vi "Convert Press. Regul. Sensor V to Bar.vi"(11 "V. Regulator Press. Sensor":dbl) -> (3 "Press. at Regulator (Bar)":dbl)   [LabVIEW 2024]
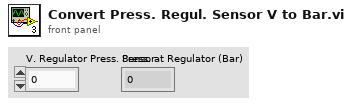
[diagram p1: front panel]
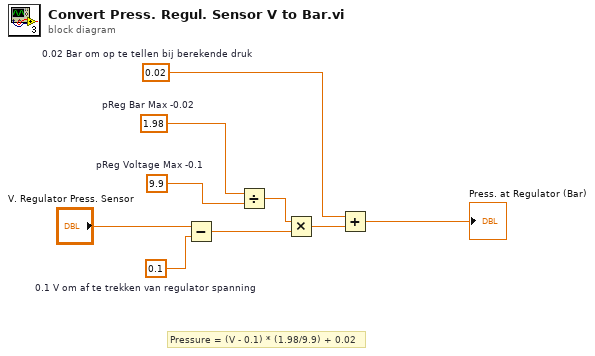
[diagram p0: block diagram]
diagram:
  w7 = 0.02  # 0.02 Bar om op te tellen bij berekende druk
  w4 = 9.9  # pReg Voltage Max -0.1
  w3 = 1.98  # pReg Bar Max -0.02
  w9 = 0.1  # 0.1 V om af te trekken van regulator spanning
  # "Pressure = (V - 0.1) * (1.98/9.9) + 0.02"
  n1 = Subtract(x="V. Regulator Press. Sensor", y=w9) -> (x-y=w2:dbl)
  n2 = Divide(x=w3, y=w4) -> (x/y=w5:dbl)
  n3 = Multiply(x=w5, y=w2) -> (x*y=w6:dbl)
  n4 = Add(x=w7, y=w6) -> (x+y=→"Press. at Regulator (Bar)":dbl)
